vi "FuncVI-DeConv.vi"(5 "InstanceRef":T2, 9 "arg list":T1[](array[typedef]) {"num" format="%.2f"}) -> (0 "error out":bool, 3 "result":T1 {"num" format="%.2f"})   [LabVIEW 2021]
doc: "::: CalcExpress Toolkit :::\nCopyright (c) 2000-2026 Konstantin Shifershteyn. All rights reserved."
uses:
  cetypes.llb/CalcExpress Function Argument Info.ctl
  cetypes.llb/CalcExpress Instance RefNum.ctl
  <vilib>/Analysis/NI_AALPro.lvlib
panel:
  in  "max arg num":i32=2
  in  "min arg num":i32=2
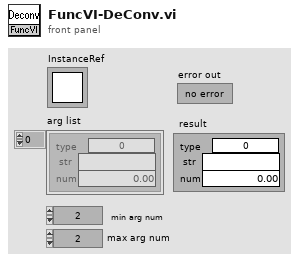
[diagram p1: front panel]
types:
  T1 = typedef "CalcExpress Function Argument Info.ctl" = cluster{"type":u32, "str":string, "num":dbl}
  T2 = typedef "CalcExpress Instance RefNum.ctl" = refnum<k1>
  T3 = enum8{"String", "DBL Number", "identifier", "1D Array of DBL", "2D Array of DBL", "CDB Number", "1D Array of CDB", "2D Array of CDB", "1D Array of String", "2D Array of String", "Unknown data type"}
  T4 = cluster{"index":i32, "type":enum8{"String", "DBL Number", "identifier", "1D Array of DBL", "2D Array of DBL", "CDB Number", "1D Array of CDB", "2D Array of CDB", "Unknown data type"}, "default num":dbl, "default str":string}[]
  T5 = cluster{"type":enum8{"String", "DBL Number", "identifier", "1D Array of DBL", "2D Array of DBL", "CDB Number", "1D Array of CDB", "2D Array of CDB", "1D Array of String", "2D Array of String", "Unknown data type"}, "data string":string, dbl}
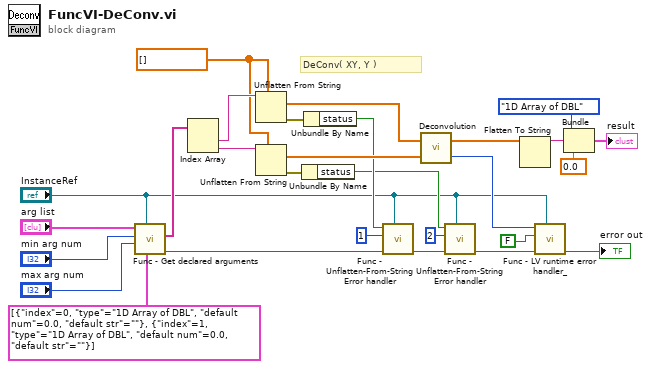
[diagram p0: block diagram]
diagram:
  w15 = dbl[] []
  # "DeConv( XY, Y )"
  n1 = call "Func - Get declared arguments.vi"("arg descriptors"=T4 [{"index"=0, "type"=enum."1D Array of DBL", "default num"=0.0, "default str"=""}, {"index"=1, "type"=enum."1D Array of DBL", "default num"=0.0, "default str"=""}] ("args descriptors"), "InstanceRef"="InstanceRef", "max arg num"="max arg num", "min arg num"="min arg num", "arg list"="arg list") -> ("error out"=w13:bool, "str list"=w18:string[])  [unwired: 3 in, 2 out]
  n2 = Index Array(array=w18) -> (element #1=w25:string, element #2=w1:string)  [unwired: 2 in]
  n3 = Unflatten From String(type=w15, binary string=w25) -> (value=w17:dbl[], error out=w2:errorcluster)  [unwired: 3 in, 1 out]
  n4 = Unflatten From String(type=w15, binary string=w1) -> (value=w16:dbl[], error out=w3:errorcluster)  [unwired: 3 in, 1 out]
  n5 = Unbundle By Name(w3) -> ("status"=w9:bool)
  n6 = Unbundle By Name(w2) -> ("status"=w10:bool)
  n7 = call "Func - Unflatten-From-String Error handler.vi"("InstanceRef"="InstanceRef", "error in"=w13, "argument number"=1, "Unflatten Error status"=w10) -> ("error out"=w12:bool)  [unwired: 5 in]
  n8 = call <vilib>:"Deconvolution.vi"("Y"=w16, "X * Y"=w17) -> ("error"=w20:i32, "X"=w24:dbl[])
  n9 = call "Func - Unflatten-From-String Error handler.vi"("InstanceRef"="InstanceRef", "error in"=w12, "argument number"=2, "Unflatten Error status"=w9) -> ("error out"=w11:bool)  [unwired: 5 in]
  n10 = Flatten To String(anything=w24) -> (data string=w22:string)  [unwired: 3 in, 2 out]
  n11 = call "Func - LV runtime error handler_.vi"("InstanceRef"="InstanceRef", "error in"=w11, "Gen CE error?"=FALSE, "LabVIEW error code"=w20) -> ("error out"=→"error out":bool)  [unwired: 7 in]
  n12 = Bundle("type"=T3."1D Array of DBL", "data string"=w22, 0.0) -> (→"result":T5)  [unwired: 1 in]
